vi "PicoScope4000aExampleAdvancedTrigger.vi"() -> ()   [LabVIEW 2010]
uses:
  shared/PicoBuffers.ctl
  PicoScope4000aLib/PicoScope4000aAnalogChannelSettings.ctl
  shared/Buffer and Transfer Settings.ctl
  shared/Acquisition Settings.ctl
panel:
  in  "Channel D Settings":T1={"Enabled"=FALSE, "Coupling"=1, "Range"=6, "Analogue Offset"=0.0, "Bandwidth Limit"=0} {"Bandwidth Limit" items=["Full", "20kHz", "100kHz", "1MHz"]; "Range" items=["10 mV", "20 mV", "50 mV", "100 mV", "200 mV", "500 mV", "1 V", "2 V", "5 V", "10 V", "20 V", "50 V ", "100 V"]; "Coupling" items=["AC", "DC"]}
  in  "Channel C Settings":T1={"Enabled"=FALSE, "Coupling"=1, "Range"=6, "Analogue Offset"=0.0, "Bandwidth Limit"=0} {"Bandwidth Limit" items=["Full", "20kHz", "100kHz", "1MHz"]; "Range" items=["10 mV", "20 mV", "50 mV", "100 mV", "200 mV", "500 mV", "1 V", "2 V", "5 V", "10 V", "20 V", "50 V ", "100 V"]; "Coupling" items=["AC", "DC"]}
  in  "roundFaster":bool
  in  "timeIntervalRequested":dbl format="%#6_6p"
  in  "Write to TDMS":bool
  out "Unit Info":T2={"Driver Version"="0", "USB Version"="0", "Hardware"="0", "Variant"="0", "Batch and Serial"="0", "Cal Date"="0", "Kernel Version"="0", "Digital HW Version"="0", "Analogue HW Version"="0", "Firmware 1"="0", "Firmware 2"="0", "Num. channels"=0}
  in  "Pulse Width Qualifier Conditions":T3 {"Channel H" items=["Don't Care", "True", "False"]; "Channel G" items=["Don't Care", "True", "False"]; "Channel F" items=["Don't Care", "True", "False"]; "Channel E" items=["Don't Care", "True", "False"]; "Aux" items=["Don't Care", "True", "False"]; "Ext" items=["Don't Care", "True", "False"]; "Channel D" items=["Don't Care", "True", "False"]; "Channel C" items=["Don't Care", "True", "False"]; "Channel B" items=["Don't Care", "True", "False"]; "Channel A" items=["Don't Care", "True", "False"]; "Condition Logic" items=["AND", "OR", "XOR"]}
  in  "Channel B Settings":T1={"Enabled"=FALSE, "Coupling"=1, "Range"=6, "Analogue Offset"=0.0, "Bandwidth Limit"=0} {"Bandwidth Limit" items=["Full", "20kHz", "100kHz", "1MHz"]; "Range" items=["10 mV", "20 mV", "50 mV", "100 mV", "200 mV", "500 mV", "1 V", "2 V", "5 V", "10 V", "20 V", "50 V ", "100 V"]; "Coupling" items=["AC", "DC"]}
  in  "Pulse Width Qualifier Settings":T4={"Direction"=2, "Lower Limit"=0, "Upper Limit"=0, "Pulse Width Type"=0} {"Pulse Width Type" items=["None", "Less Than", "Greater Than", "In Range", "Out of Range"]; "Direction" items=["Rising"=2, "Falling"=3, "Rising Lower"=7, "Above"=0, "Below"=1, "Rising or Falling"=4, "Falling Lower"=8, "Below Lower"=6, "Above Lower"=5]}
  in  "Auto Trigger (ms)":i32=1000
  in  "Channel Trigger Properties":T5={"Channel A Trigger Properties"={"thresholdUpper"=0, "thresholdUpperHysteresis"=0, "thresholdLower"=0, "thresholdLowerHysteresis"=0, "Threshold Mode"=0, "Direction"=2, "Available"=TRUE}, "Channel B Trigger Properties"={"thresholdUpper"=0, "thresholdUpperHysteresis"=0, "thresholdLower"=0, "thresholdLowerHysteresis"=0, "Threshold Mode"=0, "Direction"=2, "Available"=FALSE}, "Channel C Trigger Properties"={"thresholdUpper"=0, "thresholdUpperHysteresis"=0, "thresholdLower"=0, "thresholdLowerHysteresis"=0, "Threshold Mode"=0, "Direction"=2, "Available"=FALSE}, "Channel D Trigger Properties"={"thresholdUpper"=0, "thresholdUpperHysteresis"=0, "thresholdLower"=0, "thresholdLowerHysteresis"=0, "Threshold Mode"=0, "Direction"=2, "Available"=FALSE}, "Channel E Trigger Properties"={"thresholdUpper"=0, "thresholdUpperHysteresis"=0, "thresholdLower"=0, "thresholdLowerHysteresis"=0, "Threshold Mode"=0, "Direction"=2, "Available"=FALSE}, "Channel F Trigger Properties"={"thresholdUpper"=0, "thresholdUpperHysteresis"=0, "thresholdLower"=0, "thresholdLowerHysteresis"=0, "Threshold Mode"=0, "Direction"=2, "Available"=FALSE}, "Channel G Trigger Properties"={"thresholdUpper"=0, "thresholdUpperHysteresis"=0, "thresholdLower"=0, "thresholdLowerHysteresis"=0, "Threshold Mode"=0, "Direction"=2, "Available"=FALSE}, "Channel H Trigger Properties"={"thresholdUpper"=0, "thresholdUpperHysteresis"=0, "thresholdLower"=0, "thresholdLowerHysteresis"=0, "Threshold Mode"=0, "Direction"=2, "Available"=FALSE}} {"Channel H Trigger Properties"."Direction" items=["Above / Inside", "Below / Outside", "Rising / Enter", "Falling / Exit", "Rising or Falling / Enter or Exit", "Above Lower", "Below Lower", "Rising Lower", "Falling Lower", "Positive Runt", "Negative Runt"]; "Channel H Trigger Properties"."Threshold Mode" items=["Level", "Window"]; "Channel G Trigger Properties"."Direction" items=["Above / Inside", "Below / Outside", "Rising / Enter", "Falling / Exit", "Rising or Falling / Enter or Exit", "Above Lower", "Below Lower", "Rising Lower", "Falling Lower", "Positive Runt", "Negative Runt"]; "Channel G Trigger Properties"."Threshold Mode" items=["Level", "Window"]; "Channel F Trigger Properties"."Direction" items=["Above / Inside", "Below / Outside", "Rising / Enter", "Falling / Exit", "Rising or Falling / Enter or Exit", "Above Lower", "Below Lower", "Rising Lower", "Falling Lower", "Positive Runt", "Negative Runt"]; "Channel F Trigger Properties"."Threshold Mode" items=["Level", "Window"]; "Channel E Trigger Properties"."Direction" items=["Above / Inside", "Below / Outside", "Rising / Enter", "Falling / Exit", "Rising or Falling / Enter or Exit", "Above Lower", "Below Lower", "Rising Lower", "Falling Lower", "Positive Runt", "Negative Runt"]; "Channel E Trigger Properties"."Threshold Mode" items=["Level", "Window"]; "Channel D Trigger Properties"."Direction" items=["Above / Inside", "Below / Outside", "Rising / Enter", "Falling / Exit", "Rising or Falling / Enter or Exit", "Above Lower", "Below Lower", "Rising Lower", "Falling Lower", "Positive Runt", "Negative Runt"]; "Channel D Trigger Properties"."Threshold Mode" items=["Level", "Window"]; "Channel C Trigger Properties"."Direction" items=["Above / Inside", "Below / Outside", "Rising / Enter", "Falling / Exit", "Rising or Falling / Enter or Exit", "Above Lower", "Below Lower", "Rising Lower", "Falling Lower", "Positive Runt", "Negative Runt"]; "Channel C Trigger Properties"."Threshold Mode" items=["Level", "Window"]; "Channel B Trigger Properties"."Direction" items=["Above / Inside", "Below / Outside", "Rising / Enter", "Falling / Exit", "Rising or Falling / Enter or Exit", "Above Lower", "Below Lower", "Rising Lower", "Falling Lower", "Positive Runt", "Negative Runt"]; "Channel B Trigger Properties"."Threshold Mode" items=["Level", "Window"]; "Channel A Trigger Properties"."Direction" items=["Above / Inside", "Below / Outside", "Rising / Enter", "Falling / Exit", "Rising or Falling / Enter or Exit", "Above Lower", "Below Lower", "Rising Lower", "Falling Lower", "Positive Runt", "Negative Runt"]; "Channel A Trigger Properties"."Threshold Mode" items=["Level", "Window"]}
  in  "Trigger Conditions":T6={"Channel A"=1, "Channel B"=0, "Channel C"=0, "Channel D"=0, "Channel E"=0, "Channel F"=0, "Channel G"=0, "Channel H"=0, "Ext"=0, "Aux"=0, "PWQ"=0, "Condition Logic"=0} {"Channel H" items=["Don't Care", "True", "False"]; "Channel G" items=["Don't Care", "True", "False"]; "Channel F" items=["Don't Care", "True", "False"]; "Channel E" items=["Don't Care", "True", "False"]; "PWQ" items=["Don't Care", "True", "False"]; "Aux" items=["Don't Care", "True", "False"]; "Ext" items=["Don't Care", "True", "False"]; "Channel D" items=["Don't Care", "True", "False"]; "Channel C" items=["Don't Care", "True", "False"]; "Channel B" items=["Don't Care", "True", "False"]; "Channel A" items=["Don't Care", "True", "False"]; "Condition Logic" items=["AND", "OR", "XOR"]}
  in  "Resolution":u32(ring)=1 items=["8-bit", "12-bit", "14-bit"]
  out "overflow":i16 format="%08b"
  in  "Apply Settings":bool
  in  "Channel A Settings":T1={"Enabled"=TRUE, "Coupling"=1, "Range"=6, "Analogue Offset"=0.0, "Bandwidth Limit"=0} {"Bandwidth Limit" items=["Full", "20kHz", "100kHz", "1MHz"]; "Range" items=["10 mV", "20 mV", "50 mV", "100 mV", "200 mV", "500 mV", "1 V", "2 V", "5 V", "10 V", "20 V", "50 V ", "100 V"]; "Coupling" items=["AC", "DC"]}
  out "USB 3.0 device on non-USB 3.0 Port":bool
  out "USB Powered":bool=TRUE
  out "error out":errorcluster
  in  "Data file":path=path "PicoScope4000aExampleAdvancetrigger Data"
  in  "Buffer and Transfer Settings":T7={"startIndex"=0, "Samples"=2000000, "Down Sample Ratio"=1, "Down-Sample Mode"=0} {"Down-Sample Mode" items=["RAW none"=2147483648, "None"=0, "Aggregate"=1, "Decimate"=2, "Average"=4]; "Down Sample Ratio" step=1; "Samples" format="%_6p"}
  in  "Acquisition Settings":T8={"preTriggerSamples"=1000000, "postTriggerSamples"=1000000, "timebase"=0} {"postTriggerSamples" format="%_6p"; "preTriggerSamples" format="%_6p"}
  out "Properties Panel":T9 {"Max Total Capture Time Available (sec)" format="%.3p"; "Sample Frequency" format="%.6p"; "Sample Rate" format="%.3p"; "Max Samples Available" format="%_6p"; "Total Capture Time (sec)" format="%.3p"}
  in  "stop":bool
  out "Analog Channels":cluster{i32, dbl, "Data":dbl[]}[](graph)
  in  "Serial Number":string
  in  "Use Serial Number":bool
  in  "error in (no error)":errorcluster
  # "Bit 0 = ChA"
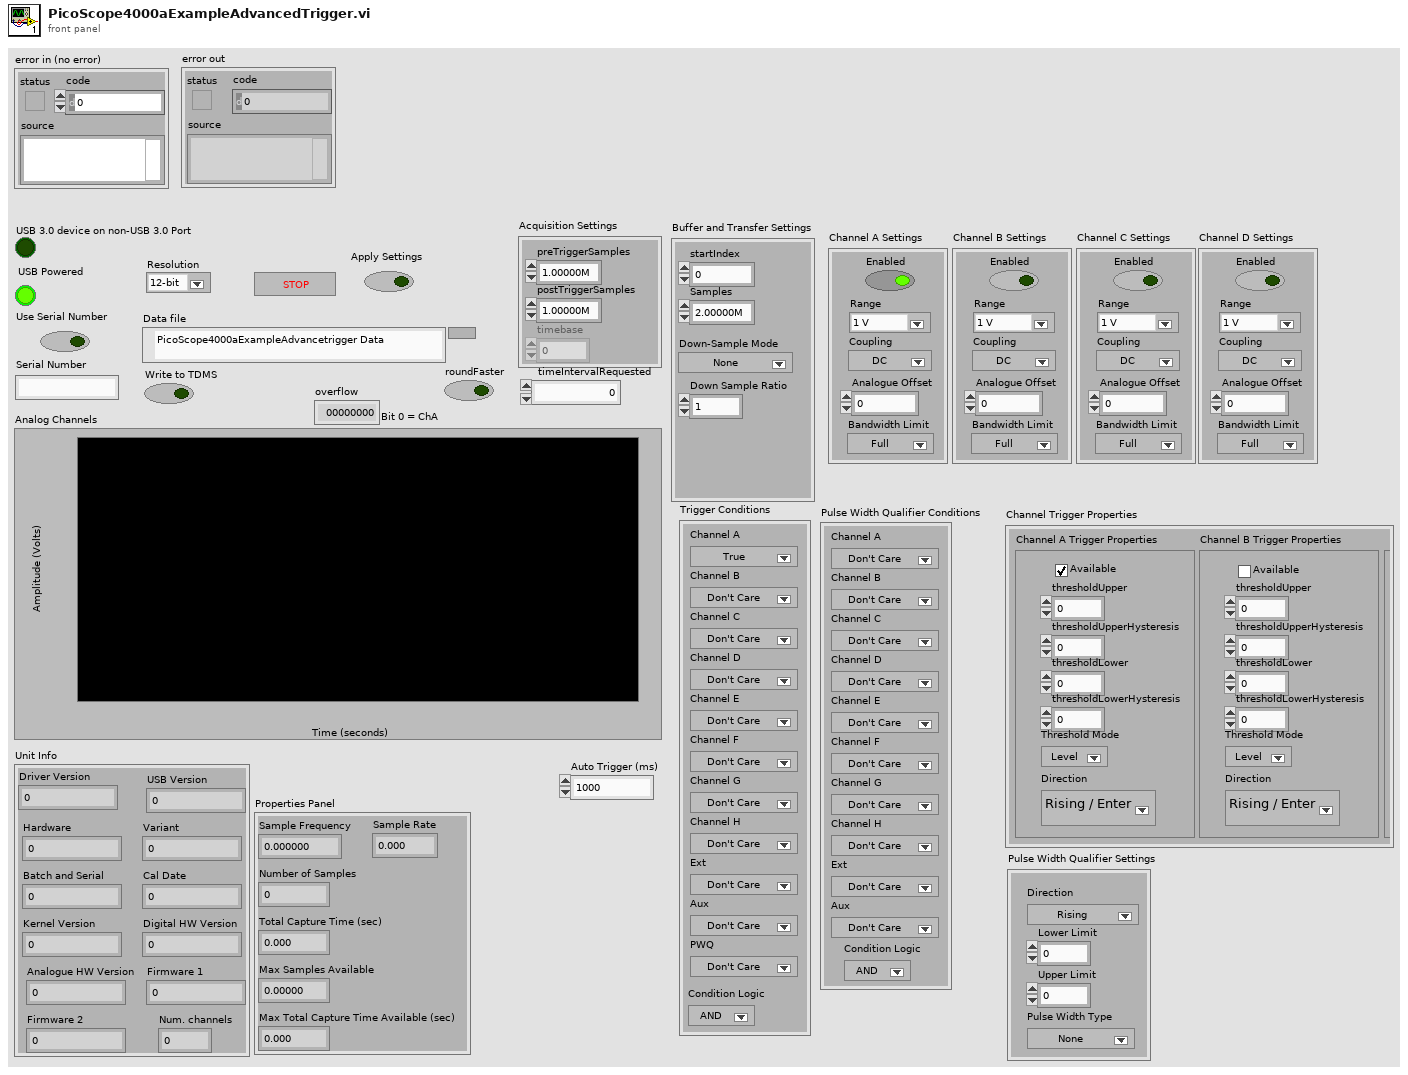
[diagram p1: front panel]
types:
  T1 = typedef "PicoScope4000aAnalogChannelSettings.ctl" = cluster{"Enabled":bool, "Coupling":i16, "Range":u32, "Analogue Offset":sgl, "Bandwidth Limit":u32}
  T2 = cluster{"Driver Version":string, "USB Version":string, "Hardware":string, "Variant":string, "Batch and Serial":string, "Cal Date":string, "Kernel Version":string, "Digital HW Version":string, "Analogue HW Version":string, "Firmware 1":string, "Firmware 2":string, "Num. channels":i16}
  T3 = cluster{"Channel A":u16, "Channel B":u16, "Channel C":u16, "Channel D":u16, "Channel E":u16, "Channel F":u16, "Channel G":u16, "Channel H":u16, "Ext":u16, "Aux":u16, "Condition Logic":u16}
  T4 = cluster{"Direction":u32, "Lower Limit":u32, "Upper Limit":u32, "Pulse Width Type":u32}
  T5 = cluster{"Channel A Trigger Properties":cluster{"thresholdUpper":i16, "thresholdUpperHysteresis":u16, "thresholdLower":i16, "thresholdLowerHysteresis":u16, "Threshold Mode":i32, "Direction":i32, "Available":bool}, "Channel B Trigger Properties":cluster{"thresholdUpper":i16, "thresholdUpperHysteresis":u16, "thresholdLower":i16, "thresholdLowerHysteresis":u16, "Threshold Mode":i32, "Direction":i32, "Available":bool}, "Channel C Trigger Properties":cluster{"thresholdUpper":i16, "thresholdUpperHysteresis":u16, "thresholdLower":i16, "thresholdLowerHysteresis":u16, "Threshold Mode":i32, "Direction":i32, "Available":bool}, "Channel D Trigger Properties":cluster{"thresholdUpper":i16, "thresholdUpperHysteresis":u16, "thresholdLower":i16, "thresholdLowerHysteresis":u16, "Threshold Mode":i32, "Direction":i32, "Available":bool}, "Channel E Trigger Properties":cluster{"thresholdUpper":i16, "thresholdUpperHysteresis":u16, "thresholdLower":i16, "thresholdLowerHysteresis":u16, "Threshold Mode":i32, "Direction":i32, "Available":bool}, "Channel F Trigger Properties":cluster{"thresholdUpper":i16, "thresholdUpperHysteresis":u16, "thresholdLower":i16, "thresholdLowerHysteresis":u16, "Threshold Mode":i32, "Direction":i32, "Available":bool}, "Channel G Trigger Properties":cluster{"thresholdUpper":i16, "thresholdUpperHysteresis":u16, "thresholdLower":i16, "thresholdLowerHysteresis":u16, "Threshold Mode":i32, "Direction":i32, "Available":bool}, "Channel H Trigger Properties":cluster{"thresholdUpper":i16, "thresholdUpperHysteresis":u16, "thresholdLower":i16, "thresholdLowerHysteresis":u16, "Threshold Mode":i32, "Direction":i32, "Available":bool}}
  T6 = cluster{"Channel A":u16, "Channel B":u16, "Channel C":u16, "Channel D":u16, "Channel E":u16, "Channel F":u16, "Channel G":u16, "Channel H":u16, "Ext":u16, "Aux":u16, "PWQ":u16, "Condition Logic":u16}
  T7 = typedef "Buffer and Transfer Settings.ctl" = cluster{"startIndex":u64, "Samples":u64, "Down Sample Ratio":u64, "Down-Sample Mode":u32}
  T8 = typedef "Acquisition Settings.ctl" = cluster{"preTriggerSamples":u64, "postTriggerSamples":u64, "timebase":u32}
  T9 = cluster{"Sample Frequency":dbl, "Sample Rate":dbl, "Max Samples Available":u64, "Number of Samples":u64, "Total Capture Time (sec) ":dbl, "Max Total Capture Time Available (sec)":dbl}
  T10 = typedef "PicoBuffers.ctl" = cluster{"Max Buffer Pointers":u64[][][], "Min Buffer Pointers":u64[][][], "StreamingDataInfo":cluster{"Channel":u32, "Down-Sample Mode":u32, "PICO_DATA_TYPE":enum32{"PICO_INT8_T", "PICO_INT16_T", "PICO_INT32_T", "PICO_UINT32_T", "PICO_INT64_T", ""}, "Samples":i32, "bufferIndex":u64, "startIndex":i32, "overflow":i16}[][]}
  T11 = enum16{"open", "open or create", "create or replace", "create", "open (read-only)"}
  T12 = cluster{"Channel A Buffer":i16[], "Channel B Buffer":i16[], "Channel C Buffer":i16[], "Channel D Buffer":i16[], "Channel E Buffer":i16[], "Channel F Buffer":i16[], "Channel G Buffer":i16[], "Channel H Buffer":i16[], "Port 0 Buffer":i16[], "Port 1 Buffer":i16[]}[]
  T13 = cluster{"Channel A Buffer":i16[], "Channel B Buffer":i16[], "Channel C Buffer":i16[], "Channel D Buffer":i16[], "Channel E Buffer":i16[], "Channel F Buffer":i16[], "Channel G Buffer":i16[], "Channel H Buffer":i16[], "Port 0 Buffer":i16[], "Port 1 Buffer":i16[]}
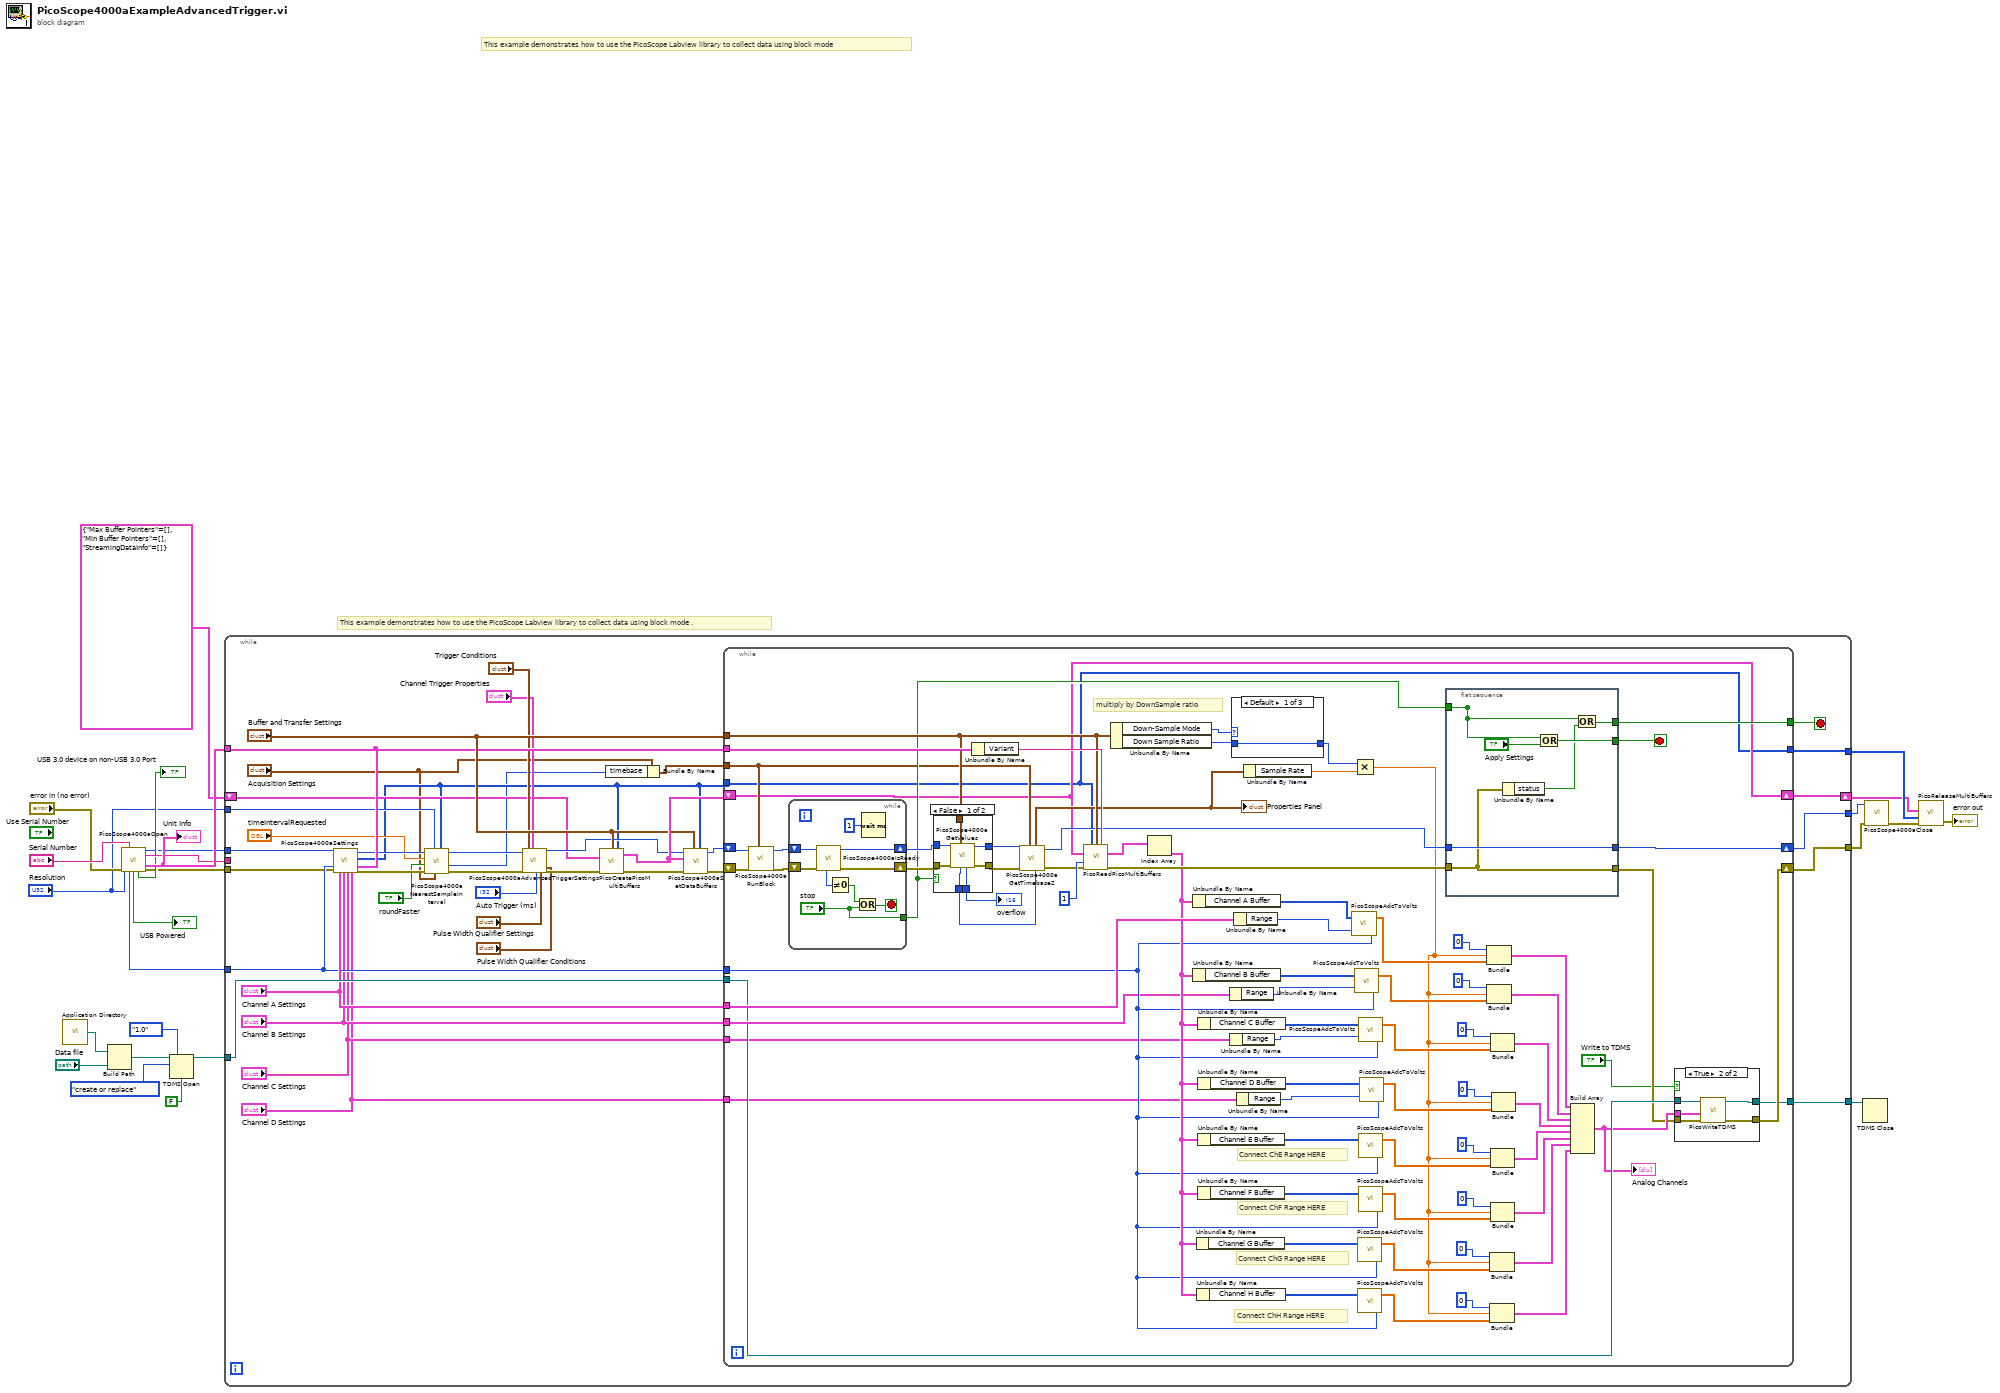
[diagram p0: block diagram]
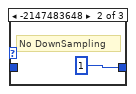
[diagram p4: hidden frame]
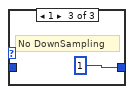
[diagram p5: hidden frame]
diagram:
  # "This example demonstrates how to use the PicoScope Labview library to collect data using block mode ."
  # "This example demonstrates how to use the PicoScope Labview library to collect data using block mode"
  n1 = call <vilib>:"Application Directory.vi"() -> ("Application Directory"=w19:path)
  n2 = Build Path(base path=w19, name or relative path="Data file") -> (appended path=w20:path)
  n3 = call "PicoScope4000aOpen.vi"("Serial Number"="Serial Number", "Resolution"="Resolution", "error in (no error)"="error in (no error)") -> ("handle"=w9:i16, "Pico 4000a Units"=w12:string, "Unit Info"=w13:T2, "Max ADC value"=w15:i16, "USB powered"=→"USB Powered":bool, "USB 3.0 on non-USB 3.0 port"=→"USB 3.0 device on non-USB 3.0 Port":bool, "error out"=w4:errorcluster)  [unwired: 5 in, 1 out]
  "Unit Info" <- w13
  n4 = TDMS Open(6:FALSE ("disable buffering? (T)"), 7:enum16{"1.0", "2.0"}."1.0" ("file format version (2.0)"), 10:T11."create or replace" ("operation (0:open)"), 11:w20) -> (3:w17:refnum<k34>)  [unwired: 2 in, 1 out]
  n5 = while {
    tunnel: w12 -> [_]
    tunnel: w15 -> [w60]
    tunnel: [w39] -> w25
    tunnel: [w58] -> w18
    tunnel: w17 -> [w62]
    tunnel: w9 -> [w43]
    tunnel: [w59] -> w7
    tunnel: [w56] -> w14
    tunnel: w13 -> [w52]
    tunnel: w4 -> [w42]
    shift-right: [w40] -> w2
    shift-left: T10 {"Max Buffer Pointers"=[], "Min Buffer Pointers"=[], "StreamingDataInfo"=[]} ("Data Pointers") -> [w41]
    tunnel: "Resolution" -> [w34]
    stop <- w57 stop-if-true
    n6 = call "PicoScope4000aSettings.vi"("handle in"=w43, "Max ADC value"=w60, "error in"=w42, "Channel A Settings"="Channel A Settings", "Channel B Settings"="Channel B Settings", "Channel C Settings"="Channel C Settings", "Channel D Settings"="Channel D Settings", "Unit Info"=w52) -> ("handle out"=w36:i16, "Enabled array"=w32:i16[], "error out"=w38:errorcluster)  [unwired: 9 in]
    n7 = call "PicoScope4000aNearestSampleInterval.vi"("Enabled array"=w32, "Acquisition Settings"="Acquisition Settings", "Resolution"=w34, "error in (no error)"=w38, "roundFaster"="roundFaster", "timeIntervalRequested"="timeIntervalRequested", "handle in"=w36) -> ("error out"=w37:errorcluster, "timebase"=w29:u32, "handle out"=w35:i16)  [unwired: 1 in, 1 out]
    n8 = call "PicoScope4000aAdvancedTriggerSettings.vi"("handle in"=w35, "error in"=w37, "Trigger Conditions"="Trigger Conditions", "Channel Trigger Properties"="Channel Trigger Properties", "Auto Trigger (ms)"="Auto Trigger (ms)", "Pulse Width Qualifier Conditions"="Pulse Width Qualifier Conditions", "Pulse Width Qualifier Settings"="Pulse Width Qualifier Settings") -> ("handle out"=w50:i16, "error out"=w51:errorcluster)  [unwired: 11 in]
    n9 = call "PicoCreatePicoMultiBuffers.vi"("Buffer and Transfer Settings"="Buffer and Transfer Settings", "enabled array"=w32, "Data Pointers In"=w41, "error in (no error)"=w51) -> ("Data Pointers"=w63:T10, "error out"=w64:errorcluster)  [unwired: 10 in]
    n10 = Bundle By Name(cluster="Acquisition Settings", "timebase"=w29) -> (w30:T8)
    n11 = call "PicoScope4000aSetDataBuffers.vi"("enabled array"=w32, "Buffer and Transfer Settings"="Buffer and Transfer Settings", "error in (no error)"=w64, "Data Pointers In"=w63, "handle in"=w50) -> ("error out"=w55:errorcluster, "handle out"=w54:i16)  [unwired: 5 in]
    n12 = while {
      tunnel: "Buffer and Transfer Settings" -> [w107]
      tunnel: w32 -> [w69]
      tunnel: "Channel A Settings" -> [w137]
      tunnel: w30 -> [w98]
      tunnel: w60 -> [w84]
      tunnel: w52 -> [w134]
      tunnel: [w114] -> w57
      shift-right: [w73] -> w59
      shift-left: w55 -> [w108]
      shift-right: [w112] -> w56
      shift-left: w54 -> [w109]
      tunnel: w62 -> [w76]
      tunnel: [w72] -> w58
      tunnel: "Channel B Settings" -> [w77]
      shift-right: [w70] -> w40
      shift-left: w63 -> [w70]
      tunnel: [w69] -> w39
      tunnel: "Channel C Settings" -> [w66]
      tunnel: "Channel D Settings" -> [w65]
      stop <- w113 stop-if-true
      # "Connect ChH Range HERE"
      # "Connect ChG Range HERE"
      # "Connect ChF Range HERE"
      # "Connect ChE Range HERE"
      # "multiply by DownSample ratio"
      n13 = call "PicoScope4000aRunBlock.vi"("Acquisition Settings"=w98, "error in (no error)"=w108, "handle in"=w109) -> ("error out"=w139:errorcluster, "handle out"=w138:i16)  [unwired: 5 in, 2 out]
      n14 = while {
        shift-right: [w174] -> w110
        shift-left: w139 -> [w175]
        shift-right: [w173] -> w111
        shift-left: w138 -> [w172]
        tunnel: ["stop"] -> w106
        stop <- w169 stop-if-true
        n15 = call "PicoScope4000aIsReady.vi"("error in (no error)"=w175, "handle in"=w172) -> ("error out"=w174:errorcluster, "handle out"=w173:i16, "ready"=w171:i16)  [unwired: 7 in]
        n16 = Not Equal To 0?(x=w171) -> (x != 0?=w170:bool)
        n17 = Or(x=w170, y="stop") -> (x .or. y?=w169:bool)
        n18 = Wait (ms)(milliseconds to wait=u32 1) -> ()  [unwired: 1 out]
      }
      n19 = case shown="False" w106 {
        tunnel: w110 -> [w157 w158]
        tunnel: w111 -> [w156 w159]
        tunnel: [w155 w159] -> w100
        tunnel: [w154 w158] -> w101
        tunnel: w107 -> [w153 _]
        tunnel: [w152 _] -> w105
        tunnel: [w151 _] -> w104
        frame False {
          n20 = call "PicoScope4000aGetValues.vi"("Buffer and Transfer Settings"=w153, "error in (no error)"=w157, "handle in"=w156) -> ("error out"=w154:errorcluster, "handle out"=w155:i16, "overflow"=w152:i16, "noOfSamples"=w151:u64)  [unwired: 5 in]
        }
        frame True {
        }
      }
      "overflow" <- w105
      n21 = Unbundle By Name(w134) -> ("Variant"=w135:string)
      n22 = call "PicoScope4000aGetTimebase2.vi"("Number of Samples"=w104, "Acquisition Settings"=w98, "error in (no error)"=w101, "handle in"=w100) -> ("error out"=w102:errorcluster, "handle out"=w99:i16, "Properties Panel"=w103:T9)  [unwired: 5 in]
      "Properties Panel" <- w103
      n23 = call "PicoReadPicoMultiBuffers.vi"("enabled array"=w69, "Buffer and Transfer Settings"=w107, "Variant"=w135, "Data Pointers"=w70, "No of Buffers"=1, "error in (no error)"=w102) -> ("MultiBuffers (Max or non-aggregated)"=w143:T12, "error out"=w115:errorcluster)  [unwired: 7 in, 1 out]
      n24 = Unbundle By Name(w107) -> ("Down-Sample Mode"=w141:u32, "Down Sample Ratio"=w142:u64)
      n25 = Index Array(array=w143) -> (element=w85:T13)  [unwired: 1 in]
      n26 = Unbundle By Name(w85) -> ("Channel A Buffer"=w124:i16[])
      n27 = Unbundle By Name(w85) -> ("Channel B Buffer"=w129:i16[])
      n28 = Unbundle By Name(w85) -> ("Channel G Buffer"=w90:i16[])
      n29 = Unbundle By Name(w85) -> ("Channel H Buffer"=w87:i16[])
      n30 = Unbundle By Name(w85) -> ("Channel C Buffer"=w122:i16[])
      n31 = Unbundle By Name(w85) -> ("Channel D Buffer"=w118:i16[])
      n32 = Unbundle By Name(w85) -> ("Channel E Buffer"=w96:i16[])
      n33 = Unbundle By Name(w85) -> ("Channel F Buffer"=w93:i16[])
      n34 = Unbundle By Name(w77) -> ("Range"=w78:u32)
      n35 = Unbundle By Name(w66) -> ("Range"=w68:u32)
      n36 = case shown="Default" w141 {
        tunnel: [w176 u64 1 ("Down Sample Ratio") u64 1 ("Down Sample Ratio")] -> w140
        tunnel: w142 -> [w176 _ _]
        frame Default {
        }
        frame -2147483648 {
          # "No DownSampling"
        }
        frame 1 {
          # "No DownSampling"
        }
      }
      n37 = Unbundle By Name(w137) -> ("Range"=w131:u32)
      n38 = Unbundle By Name(w65) -> ("Range"=w67:u32)
      n39 = Unbundle By Name(w103) -> ("Sample Rate"=w136:dbl)
      n40 = call "PicoScopeAdcToVolts.vi"("Max_adc"=w84, "Range Index"=w131, "Data"=w124) -> ("Data"=w125:dbl[])
      n41 = Multiply(x=w140, y=w136) -> (x*y=w82:dbl)
      n42 = call "PicoScopeAdcToVolts.vi"("Max_adc"=w84, "Range Index"=w78, "Data"=w129) -> ("Data"=w128:dbl[])
      n43 = call "PicoScopeAdcToVolts.vi"("Max_adc"=w84, "Data"=w90) -> ("Data"=w89:dbl[])  [unwired: 1 in]
      n44 = call "PicoScopeAdcToVolts.vi"("Max_adc"=w84, "Data"=w87) -> ("Data"=w86:dbl[])  [unwired: 1 in]
      n45 = call "PicoScopeAdcToVolts.vi"("Max_adc"=w84, "Range Index"=w68, "Data"=w122) -> ("Data"=w121:dbl[])
      n46 = call "PicoScopeAdcToVolts.vi"("Max_adc"=w84, "Data"=w96) -> ("Data"=w95:dbl[])  [unwired: 1 in]
      n47 = call "PicoScopeAdcToVolts.vi"("Max_adc"=w84, "Data"=w93) -> ("Data"=w92:dbl[])  [unwired: 1 in]
      n48 = call "PicoScopeAdcToVolts.vi"("Max_adc"=w84, "Range Index"=w67, "Data"=w118) -> ("Data"=w117:dbl[])
      n49 = flat-sequence {
        tunnel: [w166] -> w113
        tunnel: [w160] -> _
        tunnel: [w163] -> w114
        tunnel: w99 -> [w162]
        tunnel: [w162] -> w112
        tunnel: w115 -> [w161]
        tunnel: [w161] -> w74
        tunnel: w106 -> [w160]
        frame #0 {
          n50 = Unbundle By Name(w161) -> ("status"=w164:bool)
          n51 = Or(x=w160, y="Apply Settings") -> (x .or. y?=w166:bool)
          n52 = Or(x=w160, y=w164) -> (x .or. y?=w163:bool)
        }
      }
      n53 = Bundle(0, w82, "Data"=w125) -> (w127:cluster{i32, dbl, "Data":dbl[]})  [unwired: 1 in]
      n54 = Bundle(0, w82, "Data"=w128) -> (w126:cluster{i32, dbl, "Data":dbl[]})  [unwired: 1 in]
      n55 = Bundle(0, w82, "Data"=w89) -> (w80:cluster{i32, dbl, "Data":dbl[]})  [unwired: 1 in]
      n56 = Bundle(0, w82, "Data"=w86) -> (w79:cluster{i32, dbl, "Data":dbl[]})  [unwired: 1 in]
      n57 = Bundle(0, w82, "Data"=w121) -> (w120:cluster{i32, dbl, "Data":dbl[]})  [unwired: 1 in]
      n58 = Bundle(0, w82, "Data"=w95) -> (w83:cluster{i32, dbl, "Data":dbl[]})  [unwired: 1 in]
      n59 = Bundle(0, w82, "Data"=w92) -> (w81:cluster{i32, dbl, "Data":dbl[]})  [unwired: 1 in]
      n60 = Bundle(0, w82, "Data"=w117) -> (w116:cluster{i32, dbl, "Data":dbl[]})  [unwired: 1 in]
      n61 = Build Array(w127, w126, w120, w116, w83, w81, w80, w79) -> (w75:cluster{i32, dbl, "Data":dbl[]}[])
      "Analog Channels" <- w75
      n62 = case shown="True" "Write to TDMS" {
        tunnel: w75 -> [_ w150]
        tunnel: w76 -> [w144 w149]
        tunnel: w74 -> [w145 w148]
        tunnel: [w145 w147] -> w73
        tunnel: [w144 w146] -> w72
        frame False {
        }
        frame True {
          n63 = call "PicoWriteTDMS.vi"("error in (no error)"=w148, "Analog Channels"=w150, "Refnum in"=w149) -> ("error out"=w147:errorcluster, "Refnum out"=w146:refnum<k34>)  [unwired: 7 in]
        }
      }
    }
  }
  n64 = TDMS Close(11:w18) -> ()  [unwired: 1 in, 2 out]
  n65 = call "PicoScope4000aClose.vi"("error in (no error)"=w7, "handle in"=w14) -> ("error out"=w6:errorcluster)  [unwired: 7 in, 1 out]
  n66 = call "PicoReleaseMultiBuffers.vi"("error in (no error)"=w6, "Enabled array"=w25, "Data Pointers"=w2) -> ("error out"=→"error out":errorcluster)  [unwired: 7 in, 1 out]
